vi "Get Dependencies.vi"(8 "error in":errorcluster, 9 "Entire Hierarchy":bool, 10 "File Path":path, 11 "ILV File Creator in":refnum<class "ILV File Creator.lvclass">) -> (0 "error out":errorcluster, 2 "Dependencies":path[](array[path]), 3 "ILV File Creator out":refnum<class "ILV File Creator.lvclass">)   [LabVIEW 2026, in "ILV File Creator.lvclass"]
doc: "This VI determines dependencies of a LabVIEW file."
uses:
  ILV File Creator.lvclass
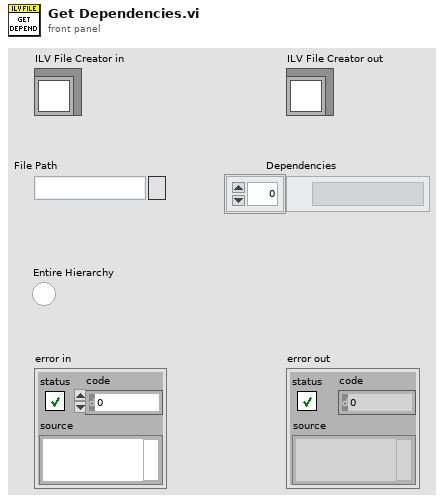
[diagram p1: front panel]
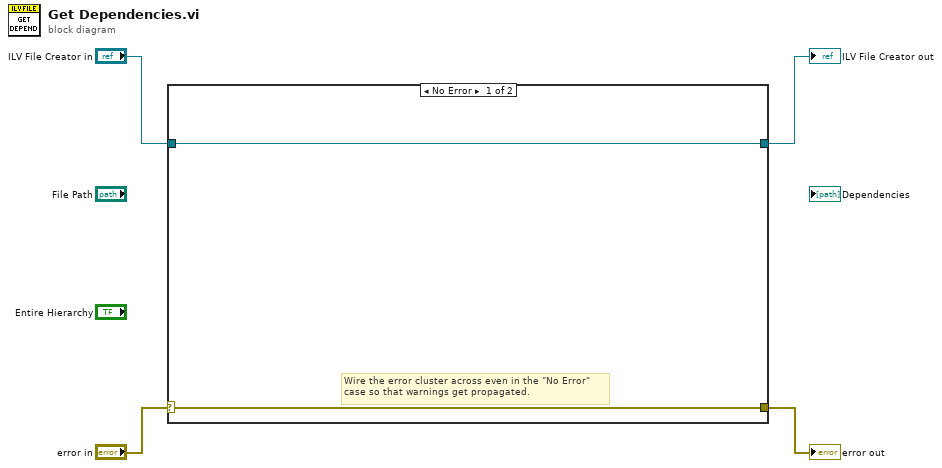
[diagram p0: block diagram]
diagram:
  n1 = case shown="No Error" "error in" {
    selector: "error in" -> [w6 w8]
    tunnel: [w6 w8] -> w3
    tunnel: [w5 w7] -> w1
    tunnel: "ILV File Creator in" -> [w5 w7]
    frame No Error {
      # "Wire the error cluster across even in the \"No Error\"\ncase so that warnings get propagated."
    }
    frame Error {
    }
  }
  "error out" <- w3
  "ILV File Creator out" <- w1
